vi "MQTT Client - Unsubscribe.vi"(0 "MQTT Session":T2, 5 "Topic Filters":string[](array[string]), 11 "error in (no error)":errorcluster) -> (4 "MQTT Session out":T2, 15 "error out":errorcluster)   [LabVIEW 2019, in "KoRE-MQTT.lvlib"]
doc: "<b>Description:</b> This VI handles the unsubscription process for an MQTT client from specified topics. It requires a reference to the MQTT session and the topic filters to which the client will unsubscribe.\n\n<b>Input Terminals:</b>\n- <b>MQTT Session [0]</b>: Reference to the active MQTT session from which the client wishes to unsubscribe.\n- <b>Topic Filters [5]</b>: Array of topic filter strings to be unsubscribed from, allowing the client to stop receiving messages from these topics. The strings must exactly match those strings used when subscribing to the topics.\n\n<b>Output Terminals:</b>\n- <b>MQTT Session out [4]</b>: Reference to the MQTT session for which the unsubscription process has been started.\n\n\nCopyright (c) 2025 KoRElibs.com\nSPDX-License-Identifier: EUPL-1.2\n\nThis VI is licensed under the European Union Public License (EUPL) Version 1.2. You may use this VI unmodified in proprietary works. If you distribute a modified version of this file, the modified file must be released under the EUPL-1.2. Full license: https://joinup.ec.europa.eu/asset/eupl/eupl/1.2/"
uses:
  KoRE-MQTT.lvlib
  TypeDefs/MQTT Client Session.ctl
  mqtt-user-property.ctl
  Private/TypeDefs/MQTT Packet - Type.ctl
  Private/MQTT Session - Get TCP Info.vi
  Private/MQTT Session - Reset Keep Alive Timer.vi
  Private/MQTT Data Stream - Write Packet.vi
panel:
  in  "User Properties (v5)":T1[](array[typedef])
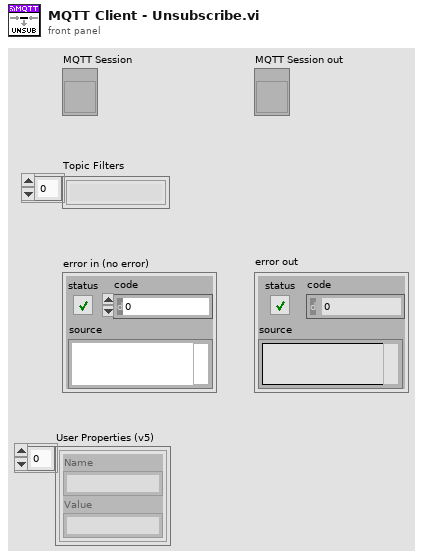
[diagram p1: front panel]
types:
  T1 = typedef "KoRE-MQTT.lvlib/mqtt-user-property.ctl" = cluster{"Name":string, "Value":string}
  T2 = typedef "KoRE-MQTT.lvlib/MQTT Client Session.ctl" = refnum<vi>
  T3 = typedef "KoRE-MQTT.lvlib/MQTT Packet - Type.ctl" = enum32{"Reserved", "CONNECT", "CONNACK", "PUBLISH", "PUBACK", "PUBREC", "PUBREL", "PUBCOMP", "SUBSCRIBE", "SUBACK", "UNSUBSCRIBE", "UNSUBACK", "PINGREQ", "PINGRESP", "DISCONNECT", "AUTH"}
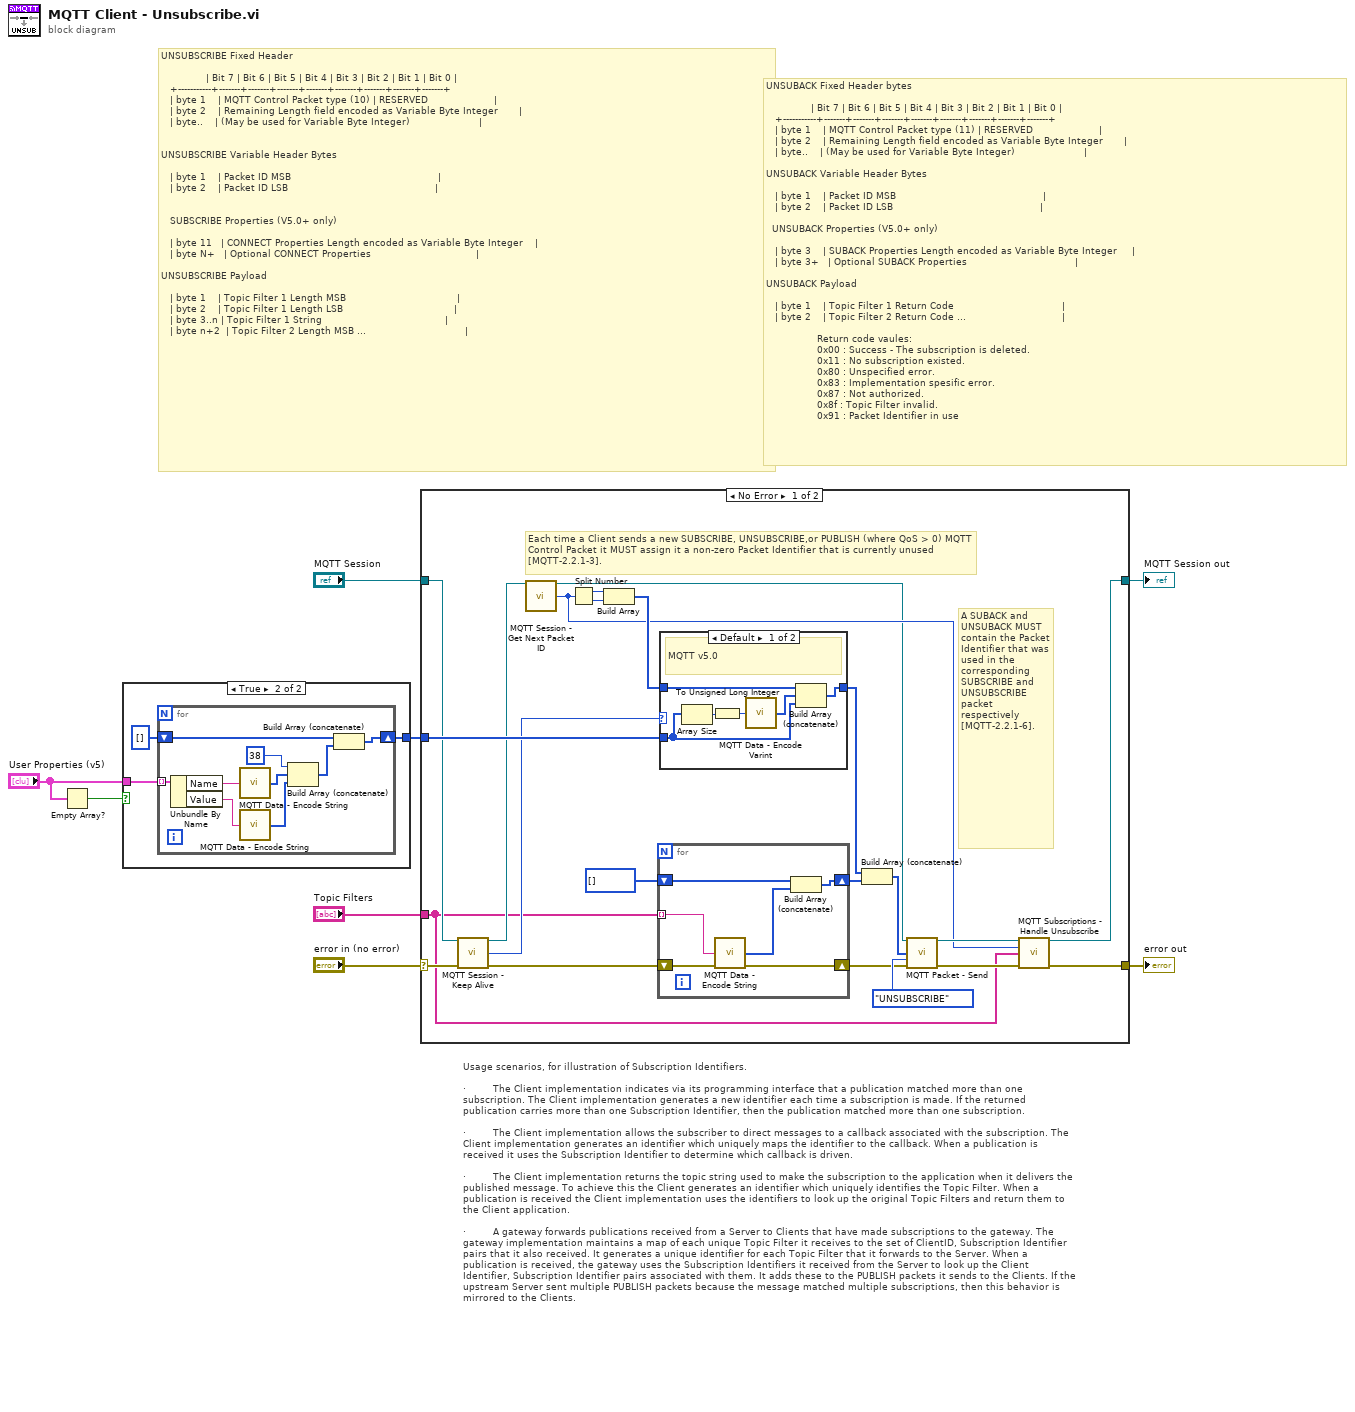
[diagram p0: block diagram]
diagram:
  # "Usage scenarios, for illustration of Subscription Identifiers.\n\n·         The Client implementation indicates via its programming interface that a publication matched more than one subscription. The Client implementation generates a new identifier each time a subscription is made. If the returned publication carries more than one Subscription Identifier, then the publication matched more than one subscription.\n\n·         The Client implementation allows the subscriber to direct messages to a callback associated with the subscription. The Client implementation generates an identifier which uniquely maps the identifier to the callback. When a publication is received it uses the Subscription Identifier to determine which callback is driven.\n\n·         The Client implementation returns the topic string used to make the subscription to the application when it delivers the published message. To achieve this the Client generates an identifier which uniquely identifies the Topic Filter. When a publication is received the Client implementation uses the identifiers to look up the original Topic Filters and return them to the Client application.\n\n·         A gateway forwards publications received from a Server to Clients that have made subscriptions to the gateway. The gateway implementation maintains a map of each unique Topic Filter it receives to the set of ClientID, Subscription Identifier pairs that it also received. It generates a unique identifier for each Topic Filter that it forwards to the Server. When a publication is received, the gateway uses the Subscription Identifiers it received from the Server to look up the Client Identifier, Subscription Identifier pairs associated with them. It adds these to the PUBLISH packets it sends to the Clients. If the upstream Server sent multiple PUBLISH packets because the message matched multiple subscriptions, then this behavior is mirrored to the Clients."
  # "UNSUBACK Fixed Header bytes\n\n               | Bit 7 | Bit 6 | Bit 5 | Bit 4 | Bit 3 | Bit 2 | Bit 1 | Bit 0 |\n   +-----------+-------+-------+-------+-------+-------+-------+-------+-------+\n   | byte 1    | MQTT Control Packet type (11) | RESERVED                      |\n   | byte 2    | Remaining Length field encoded as Variable Byte Integer       |\n   | byte..    | (May be used for Variable Byte Integer)                       | \n\nUNSUBACK Variable Header Bytes\n\n   | byte 1    | Packet ID MSB                                                 |  \n   | byte 2    | Packet ID LSB                                                 |\n\n  UNSUBACK Properties (V5.0+ only)\n\n   | byte 3    | SUBACK Properties Length encoded as Variable Byte Integer     |\n   | byte 3+   | Optional SUBACK Properties                                    |\n\nUNSUBACK Payload \n\n   | byte 1    | Topic Filter 1 Return Code                                    |\n   | byte 2    | Topic Filter 2 Return Code ...                                |\n\n                 Return code vaules: \n                 0x00 : Success - The subscription is deleted.\n                 0x11 : No subscription existed.\n                 0x80 : Unspecified error.\n                 0x83 : Implementation spesific error.\n                 0x87 : Not authorized.\n                 0x8f : Topic Filter invalid.\n                 0x91 : Packet Identifier in use"
  # "UNSUBSCRIBE Fixed Header\n\n               | Bit 7 | Bit 6 | Bit 5 | Bit 4 | Bit 3 | Bit 2 | Bit 1 | Bit 0 |\n   +-----------+-------+-------+-------+-------+-------+-------+-------+-------+\n   | byte 1    | MQTT Control Packet type (10) | RESERVED                      |\n   | byte 2    | Remaining Length field encoded as Variable Byte Integer       |\n   | byte..    | (May be used for Variable Byte Integer)                       | \n\n\nUNSUBSCRIBE Variable Header Bytes\n\n   | byte 1    | Packet ID MSB                                                 |  \n   | byte 2    | Packet ID LSB                                                 |\n\n\n   SUBSCRIBE Properties (V5.0+ only)\n\n   | byte 11   | CONNECT Properties Length encoded as Variable Byte Integer    |\n   | byte N+   | Optional CONNECT Properties                                   |\n\nUNSUBSCRIBE Payload \n\n   | byte 1    | Topic Filter 1 Length MSB                                     |\n   | byte 2    | Topic Filter 1 Length LSB                                     |\n   | byte 3..n | Topic Filter 1 String                                         |\n   | byte n+2  | Topic Filter 2 Length MSB ...                                 |"
  n1 = Empty Array?(array="User Properties (v5)") -> (empty?=w3:bool)
  n2 = case shown="True" w3 {
    tunnel: "User Properties (v5)" -> [_ w11]
    tunnel: [_ w9] -> w1
    frame False {
    }
    frame True {
      n3 = for {
        tunnel: w11 -> [w20] mode=indexing
        shift-right: [w14] -> w9
        shift-left: u8[] [] -> [w12]
        n4 = Unbundle By Name(w20) -> ("Name"=w16:string, "Value"=w15:string)
        n5 = call "MQTT Data - Encode String.vi"("String in"=w16) -> ("Bytes out"=w18:u8[])  [unwired: 13 in, 1 out]
        n6 = call "MQTT Data - Encode String.vi"("String in"=w15) -> ("Bytes out"=w17:u8[])  [unwired: 13 in, 1 out]
        n7 = Build Array (concatenate)(u8 38, w18, w17) -> (w13:u8[])
        n8 = Build Array (concatenate)(w12, w13) -> (w14:u8[])
      }
    }
  }
  n9 = case shown="No Error" "error in (no error)" {
    selector: "error in (no error)" -> [w33 w57]
    tunnel: [w25 w57] -> w7
    tunnel: "MQTT Session" -> [w35 w56]
    tunnel: "Topic Filters" -> [w29 _]
    tunnel: [w24 w56] -> w4
    tunnel: w1 -> [w38 _]
    frame No Error {
      # "A SUBACK and UNSUBACK MUST contain the Packet Identifier that was used in the corresponding SUBSCRIBE and UNSUBSCRIBE packet respectively [MQTT-2.2.1-6]."
      # "Each time a Client sends a new SUBSCRIBE, UNSUBSCRIBE,or PUBLISH (where QoS > 0) MQTT Control Packet it MUST assign it a non-zero Packet Identifier that is currently unused [MQTT-2.2.1-3]."
      n10 = call "MQTT Session - Keep Alive.vi"("mqtt ref in"=w35, "error in"=w33) -> ("mqtt ref out"=w36:T2, "Version"=w34:u8, "error out"=w32:errorcluster)  [unwired: 11 in]
      n11 = call "MQTT Session - Get Next Packet ID.vi"("MQTT_Q In in"=w36) -> ("MQTT_Q In out"=w26:T2, "PacketID"=w28:u16)  [unwired: 13 in]
      n12 = Split Number(x=w28) -> (hi(x)=w41:u8, lo(x)=w42:u8)
      n13 = Build Array(w41, w42) -> (w37:u8[])
      n14 = for {
        shift-right: [w54] -> w27
        shift-left: w32 -> [w55]
        shift-right: [w51] -> w22
        shift-left: u8[] [] -> [w52]
        tunnel: w29 -> [w50] mode=indexing
        n15 = call "MQTT Data - Encode String.vi"("String in"=w50, "error in (no error)"=w55) -> ("Bytes out"=w53:u8[], "error out"=w54:errorcluster)  [unwired: 12 in]
        n16 = Build Array (concatenate)(w52, w53) -> (w51:u8[])
      }
      n17 = case shown="Default" w34 {
        tunnel: w37 -> [w48 w49]
        tunnel: [w47 w49] -> w23
        tunnel: w38 -> [w43 _]
        frame Default {
          # "MQTT v5.0"
          n18 = Array Size(array=w43) -> (size(s)=w46:i32)
          n19 = To Unsigned Long Integer(number=w46) -> (unsigned 32bit integer=w45:u32)
          n20 = call "MQTT Data - Encode Varint.vi"("Value"=w45) -> ("encoded value"=w44:u8[])  [unwired: 14 in]
          n21 = Build Array (concatenate)(w48, w44, w43) -> (w47:u8[])
        }
        frame 3, 4 {
          # "MQTT v3.11"
        }
      }
      n22 = Build Array (concatenate)(w23, w22) -> (w21:u8[])
      n23 = call "MQTT Packet - Send.vi"("mqtt ref in"=w26, "packet data"=w21, "MessageType"=MQTT_Packet_-_Type."UNSUBSCRIBE", "error in (no error)"=w27) -> ("mqtt ref out"=w31:T2, "error out"=w30:errorcluster)  [unwired: 9 in, 1 out]
      n24 = call "MQTT Subscriptions - Handle Unsubscribe.vi"("MQTT ref in"=w31, "Packet ID"=w28, "Topic Filters"=w29, "error in"=w30) -> ("MQTT ref out"=w24:T2, "error out"=w25:errorcluster)  [unwired: 10 in]
    }
    frame Error {
    }
  }
  "error out" <- w7
  "MQTT Session out" <- w4
